vi "ecc register error code n2e.vi"(0 "number":u32 format="%0d", 1 "error in (no error)":errorcluster) -> (2 "error out":errorcluster, 3 "enum":T1)   [LabVIEW 2024, in "atsj peakcan basic.lvlib"]
uses:
  atsj peakcan basic.lvlib
  ecc register error code.ctl
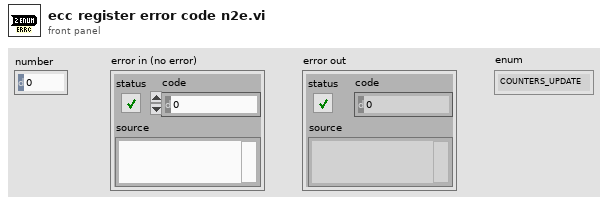
[diagram p1: front panel]
types:
  T1 = typedef "atsj peakcan basic.lvlib/ecc register error code.ctl" = enum8{"COUNTERS_UPDATE", "BIT_ERROR", "FORM_ERROR", "STUFF_ERROR", "OTHER_ERROR"}
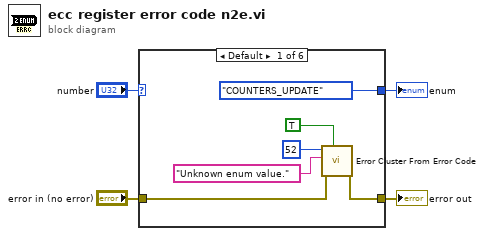
[diagram p0: block diagram]
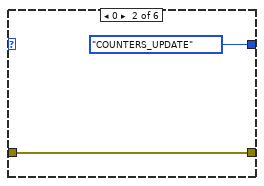
[diagram p2: hidden frame]
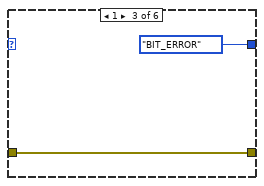
[diagram p3: hidden frame]
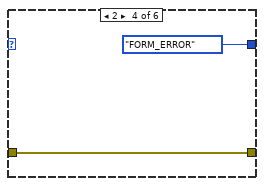
[diagram p4: hidden frame]
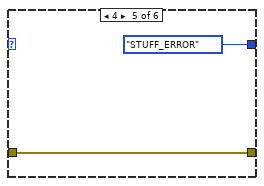
[diagram p5: hidden frame]
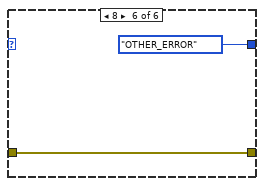
[diagram p6: hidden frame]
diagram:
  n1 = case shown="Default" "number" {
    tunnel: [ecc_register_error_code."COUNTERS_UPDATE" ecc_register_error_code."COUNTERS_UPDATE" ecc_register_error_code."BIT_ERROR" ecc_register_error_code."FORM_ERROR" ecc_register_error_code."STUFF_ERROR" ecc_register_error_code."OTHER_ERROR"] -> w3
    tunnel: "error in (no error)" -> [w6 w11 w13 w15 w17 w19]
    tunnel: [w5 w11 w13 w15 w17 w19] -> w1
    frame Default {
      n2 = call <vilib>:"Error Cluster From Error Code.vi"("show call chain? (False)"=TRUE, "error in (no error)"=w6, "error message (\"\")"="Unknown enum value.", "error code (0)"=52) -> ("error out"=w5:errorcluster)  [unwired: 5 in]
    }
    frame 0 {
    }
    frame 1 {
    }
    frame 2 {
    }
    frame 4 {
    }
    frame 8 {
    }
  }
  "enum" <- w3
  "error out" <- w1
